vi "Analog_Read.vi"(8 "error in (no error)":errorcluster, 10 "Canal":u8, 11 "VISA resource name":refnum<visa-resource-name>) -> (0 "error out":errorcluster, 2 "Out":i32, 3 "VISA resource name out":refnum<visa-resource-name>)   [LabVIEW 2026]
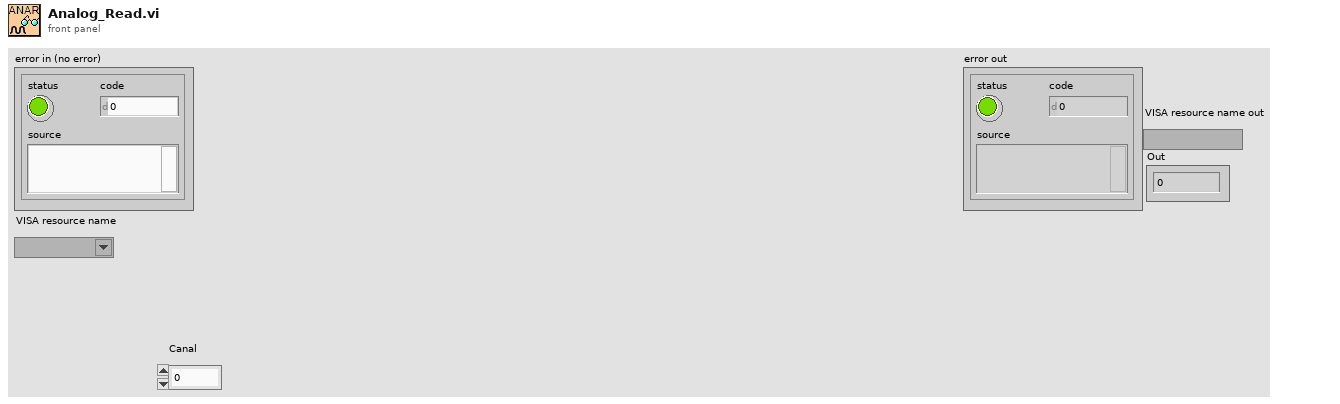
[diagram p1: front panel]
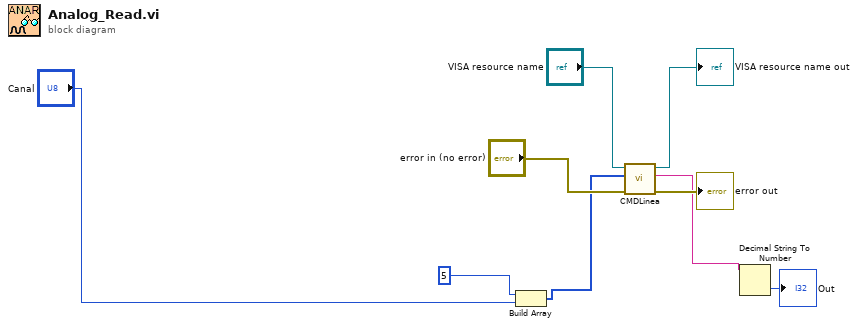
[diagram p0: block diagram]
diagram:
  n1 = Build Array(u8 5, "Canal") -> (w3:u8[])
  n2 = call "CMDLinea.vi"("error in (no error)"="error in (no error)", "Comando"=w3, "VISA resource name"="VISA resource name") -> ("error out"=→"error out":errorcluster, "respuesta"=w2:string, "VISA resource name out"=→"VISA resource name out":refnum<visa-resource-name>)  [unwired: 6 in]
  n3 = Decimal String To Number(string=w2) -> (number=→"Out":i32)  [unwired: 2 in, 1 out]
